vi "StatusStrip.vi"(8 "error in (no error)":errorcluster caption="错误输入（无错误）", 10 "VI引用":refnum<vi>, 11 "StatusStrip":refnum<k24>) -> (0 "Fail":refnum<k24>, 1 "Pass":refnum<k24>, 2 "PassY":refnum<k24>, 3 "Text":refnum<k24>)   [LabVIEW 2025]
uses:
  System.Windows.Forms
  System.Drawing
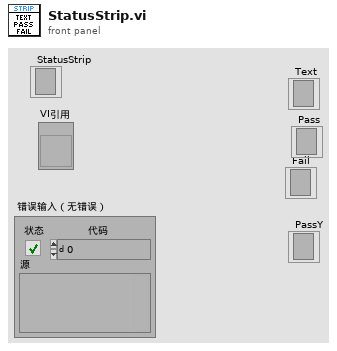
[diagram p1: front panel]
types:
  T1 = typedef "LVRectTypeDef.ctl" = cluster{"Left":i16, "Top":i16, "Right":i16, "Bottom":i16}
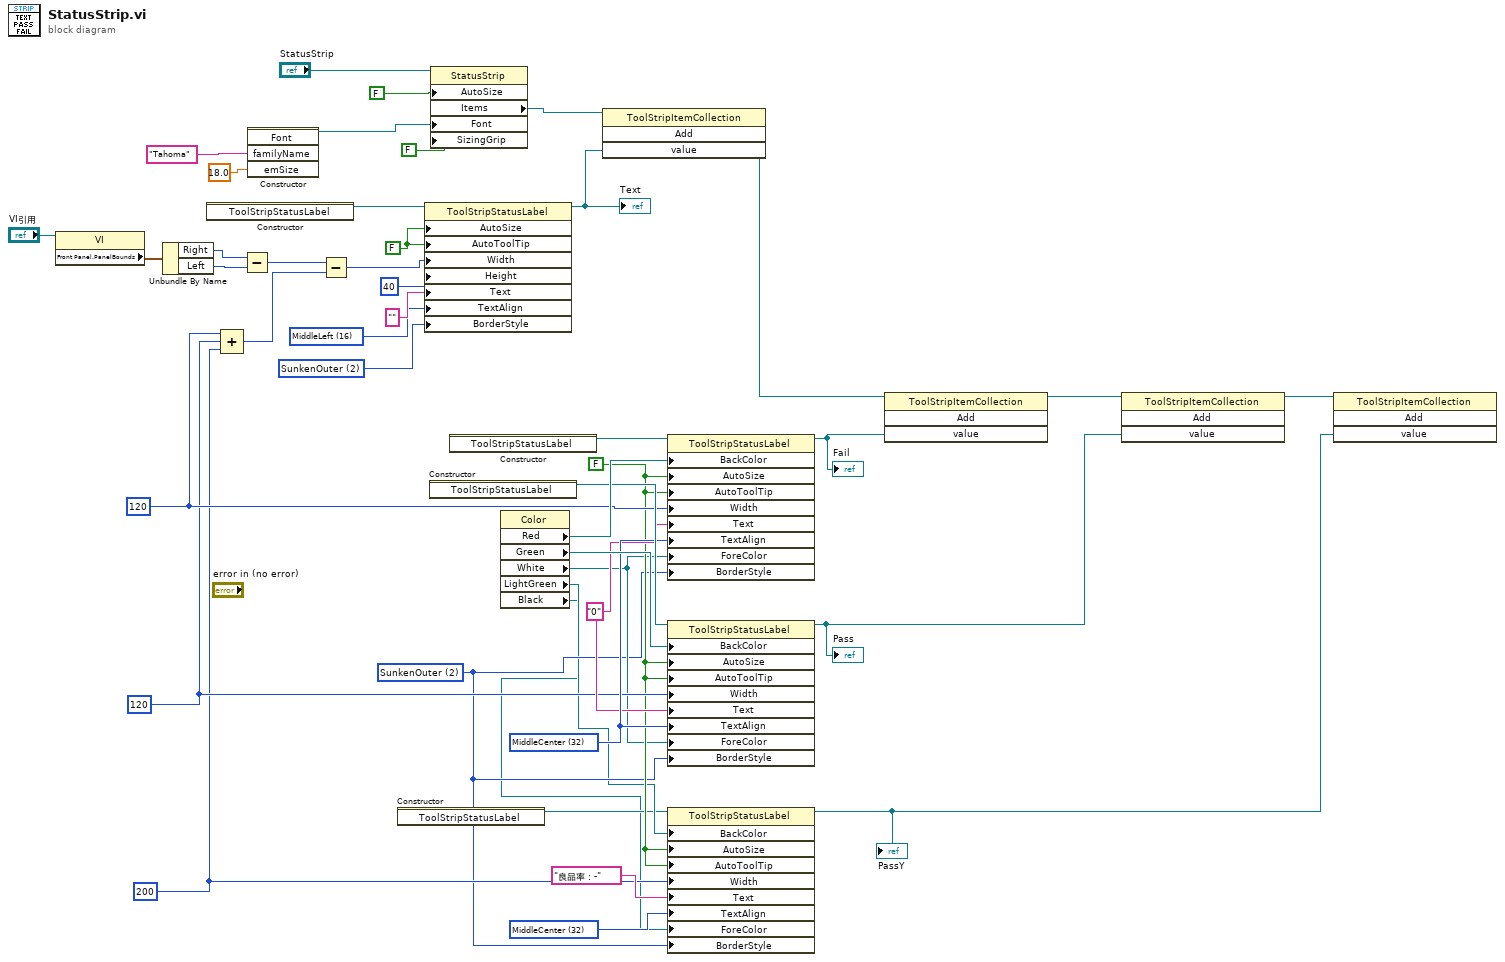
[diagram p0: block diagram]
diagram:
  w7 = 200 ("Width")
  w10 = 32 items=["TopLeft"=1, "TopCenter"=2, "TopRight"=4, "MiddleLeft"=16, "MiddleCenter"=32, "MiddleRight"=64, "BottomLeft"=256, "BottomCenter"=512, "BottomRight"=1024] ("TextAlign")
  w12 = 120 ("Width")
  w15 = 2 items=["RaisedOuter"=1, "SunkenOuter"=2, "RaisedInner"=4, "Raised"=5, "Etched"=6, "SunkenInner"=8, "Bump"=9, "Sunken"=10, "Adjust"=8192, "Flat"=16394] ("BorderStyle")
  w6 = 2 items=["RaisedOuter"=1, "SunkenOuter"=2, "RaisedInner"=4, "Raised"=5, "Etched"=6, "SunkenInner"=8, "Bump"=9, "Sunken"=10, "Adjust"=8192, "Flat"=16394] ("BorderStyle")
  w36 = 16 items=["TopLeft"=1, "TopCenter"=2, "TopRight"=4, "MiddleLeft"=16, "MiddleCenter"=32, "MiddleRight"=64, "BottomLeft"=256, "BottomCenter"=512, "BottomRight"=1024] ("TextAlign")
  w26 = 32 items=["TopLeft"=1, "TopCenter"=2, "TopRight"=4, "MiddleLeft"=16, "MiddleCenter"=32, "MiddleRight"=64, "BottomLeft"=256, "BottomCenter"=512, "BottomRight"=1024] ("TextAlign")
  w25 = "0" ("Text")
  w13 = 120 ("Width")
  w9 = FALSE ("AutoSize")
  w39 = FALSE ("AutoSize")
  n1 = property class="VI"(reference="VI引用") -> ("Front Panel.PanelBounds"=w20:T1)  [unwired: 1 in, 2 out]
  n2 = Unbundle By Name(w20) -> ("Right"=w19:i16, "Left"=w18:i16)
  n3 = constructor class="ToolStripStatusLabel"() -> (reference out=w40:refnum<k24>)  [unwired: 3 in, 2 out]
  n4 = Compound Arithmetic op=unknown(w13, w12, w7) -> (w14:i32)
  n5 = Subtract(x=w19, y=w18) -> (x-y=w17:i16)
  n6 = constructor class="Font"("familyName"="Tahoma", "emSize"=sgl 18.0) -> (reference out=w34:refnum<k24>)  [unwired: 3 in, 4 out]
  n7 = Subtract(x=w17, y=w14) -> (x-y=w16:i32)
  n8 = constructor class="ToolStripStatusLabel"() -> (reference out=w2:refnum<k24>)  [unwired: 3 in, 2 out]
  n9 = property class="ToolStripStatusLabel"(reference=w40, "AutoSize"=w39, "AutoToolTip"=w39, "Width"=w16, "Height"=40, "Text"="", "TextAlign"=w36, "BorderStyle"=w15) -> (reference out=w24:refnum<k24>)  [unwired: 1 in, 1 out]
  "Text" <- w24
  n10 = constructor class="ToolStripStatusLabel"() -> (reference out=w29:refnum<k24>)  [unwired: 3 in, 2 out]
  n11 = property class="StatusStrip"(reference="StatusStrip", "AutoSize"=FALSE, "Font"=w34, "SizingGrip"=FALSE) -> ("Items"=w35:refnum<k24>)  [unwired: 1 in, 2 out]
  n12 = constructor class="ToolStripStatusLabel"() -> (reference out=w30:refnum<k24>)  [unwired: 3 in, 2 out]
  n13 = property class="Color"() -> ("Red"=w42:refnum<k24>, "Green"=w31:refnum<k24>, "White"=w8:refnum<k24>, "LightGreen"=w5:refnum<k24>, "Black"=w1:refnum<k24>)  [unwired: 2 in, 2 out]
  n14 = invoke class="ToolStripItemCollection" method="Add"(reference=w35, "value"=w24) -> (reference out=w43:refnum<k24>)  [unwired: 2 in, 3 out]
  n15 = property class="ToolStripStatusLabel"(reference=w30, "BackColor"=w42, "AutoSize"=w9, "AutoToolTip"=w9, "Width"=w13, "Text"=w25, "TextAlign"=w26, "ForeColor"=w8, "BorderStyle"=w6) -> (reference out=w23:refnum<k24>)  [unwired: 1 in, 1 out]
  "Fail" <- w23
  n16 = property class="ToolStripStatusLabel"(reference=w29, "BackColor"=w31, "AutoSize"=w9, "AutoToolTip"=w9, "Width"=w12, "Text"=w25, "TextAlign"=w26, "ForeColor"=w8, "BorderStyle"=w6) -> (reference out=w22:refnum<k24>)  [unwired: 1 in, 1 out]
  "Pass" <- w22
  n17 = property class="ToolStripStatusLabel"(reference=w2, "BackColor"=w5, "AutoSize"=w9, "AutoToolTip"=w9, "Width"=w7, "Text"="良品率：-", "TextAlign"=w10, "ForeColor"=w1, "BorderStyle"=w6) -> (reference out=w3:refnum<k24>)  [unwired: 1 in, 1 out]
  "PassY" <- w3
  n18 = invoke class="ToolStripItemCollection" method="Add"(reference=w43, "value"=w23) -> (reference out=w41:refnum<k24>)  [unwired: 2 in, 3 out]
  n19 = invoke class="ToolStripItemCollection" method="Add"(reference=w41, "value"=w22) -> (reference out=w4:refnum<k24>)  [unwired: 2 in, 3 out]
  n20 = invoke class="ToolStripItemCollection" method="Add"(reference=w4, "value"=w3) -> ()  [unwired: 2 in, 4 out]
